vi "Native_CreateLocalVariable_v5.vi"() -> ()   [LabVIEW 2024]
panel:
  out "error out":errorcluster caption="错误输出"
  out "terminal_ids":u32[](array[numeric])
  in  "terminal_ids type":u32
  in  "write":bool
  out "local_id":u32
  in  "local_id type":u32
  in  "control_id":u32
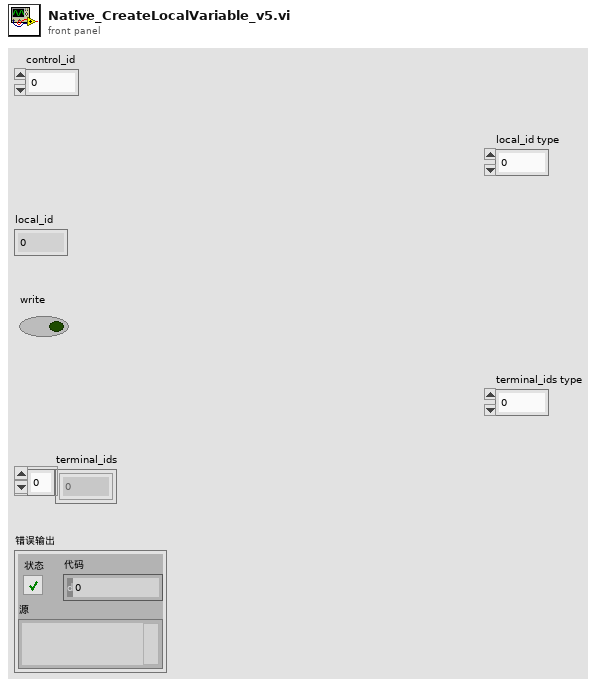
[diagram p1: front panel]
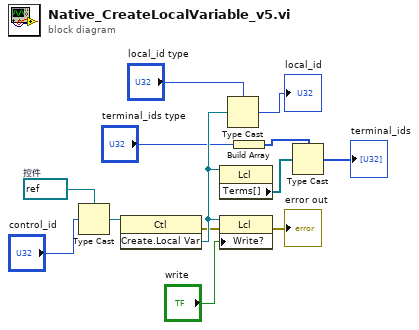
[diagram p0: block diagram]
diagram:
  w12 = refnum<vi> refnum  # 控件
  n1 = Type Cast ("强制类型转换")(type=w12, x="control_id") -> (*(type *) &x=w11:refnum<vi>)
  n2 = invoke class="Ctl" method="Create.Local Var"(reference=w11) -> (error out=w6:errorcluster, "Create Local"=w10:refnum<vi>)  [unwired: 2 in, 1 out]
  n3 = property on="属性节点" class="Lcl"(reference=w10) -> ("Terms[]"=w5:refnum<vi>[])  [unwired: 1 in, 2 out]
  n4 = property on="属性节点" class="Lcl"(reference=w10, error in=w6, "Write?"="write") -> (error out=→"error out":errorcluster)  [unwired: 1 out]
  n5 = Type Cast ("强制类型转换")(type="local_id type", x=w10) -> (*(type *) &x=→"local_id":u32)
  n6 = Build Array ("创建数组")("terminal_ids type") -> (w3:u32[])
  n7 = Type Cast ("强制类型转换")(type=w3, x=w5) -> (*(type *) &x=→"terminal_ids":u32[])
